vi "TreeUpdate.vi"(8 "error in":errorcluster, 11 "Data input":T1) -> (0 "error out":errorcluster, 3 "Data output":T1)   [LabVIEW 2017]
doc: "<B>This VI is used for updating tree item with Caps properties.</B>"
uses:
  Ctrl/Data.ctl
  Ctrl/Caps.ctl
  Ctrl/Property.ctl
  Ctrl/PhysicalChannel.ctl
  Ctrl/Register.ctl
  Ctrl/Bitfield.ctl
  Ctrl/Scale.ctl
  Ctrl/ScaleType.ctl
  Ctrl/Enum.ctl
  Ctrl/EnumValue.ctl
  API/Tree/SLSC Tree Control.lvlib
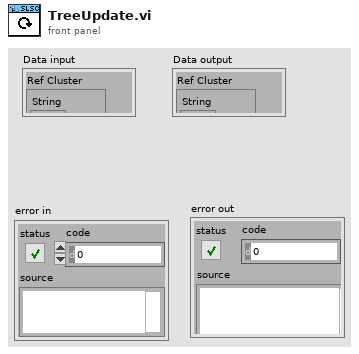
[diagram p1: front panel]
types:
  T1 = typedef "Data.ctl" = cluster{"Ref Cluster":cluster{"String":refnum<vi>, "U8":refnum<vi>, "I8":refnum<vi>, "U32":refnum<vi>, "I32":refnum<vi>, "U64":refnum<vi>, "I64":refnum<vi>, "Ring":refnum<vi>, "DBL":refnum<vi>, "Add":refnum<vi>, "Remove":refnum<vi>, "Property tree":refnum<vi>, "confirm":refnum<vi>}, "JSON Text":string, "Original JSON Text":string, "Caps":T2, "SLSC Output Tree":cluster{"Left Cell String":string, "Child Text":string[], "Child Tag":string, "Item Indent":i32, "Child Only?":bool, "Glyph Index":i32, "offline value":variant}[], "Ref Index and Control Type":cluster{"index":i32, "Datatype":string}, "Selected Type and name":cluster{"Selected Type":enum16{"Property", "Physical Channel", "Other"}, "Selected Property Name":string}, "Update whole Tree?":bool}
  T2 = typedef "Caps.ctl" = cluster{"properties":T3[], "physical channels":T4[], "registers":T5[], "scales":T7[], "enums":T9[], "productName":string}
  T3 = typedef "Property.ctl" = cluster{"name":string, "bitfield":string, "value":variant, "dataType":string, "min":variant, "max":variant, "scale":string, "access":string}
  T4 = typedef "PhysicalChannel.ctl" = cluster{"name":string, "properties":T3[]}
  T5 = typedef "Register.ctl" = cluster{"name":string, "address":i32, "size":i32, "bitfields":T6[], "initialValue":variant, "connectedProperties":string[]}
  T6 = typedef "Bitfield.ctl" = cluster{"name":string, "offset":i32, "size":i32, "signed":bool}
  T7 = typedef "Scale.ctl" = cluster{"name":string, "type":T8, "params":variant}
  T8 = typedef "ScaleType.ctl" = enum16{"NoScale", "Table", "Polynomial", "Linear"}
  T9 = typedef "Enum.ctl" = cluster{"name":string, "values":T10[]}
  T10 = typedef "EnumValue.ctl" = cluster{"name":string, "value":i32}
  T11 = cluster{"name":string, "string enums":string, "values":T10[]}[]
  T12 = cluster{"Left Cell String":string, "Child Text":string[], "Child Tag":string, "Item Indent":i32, "Child Only?":bool, "Glyph Index":i32, "offline value":variant}[]
  T13 = cluster{"Left Cell String":string, "Child Text":string[], "Child Tag":string, "Item Indent":i32, "Child Only?":bool, "Glyph Index":i32, "offline value":variant}
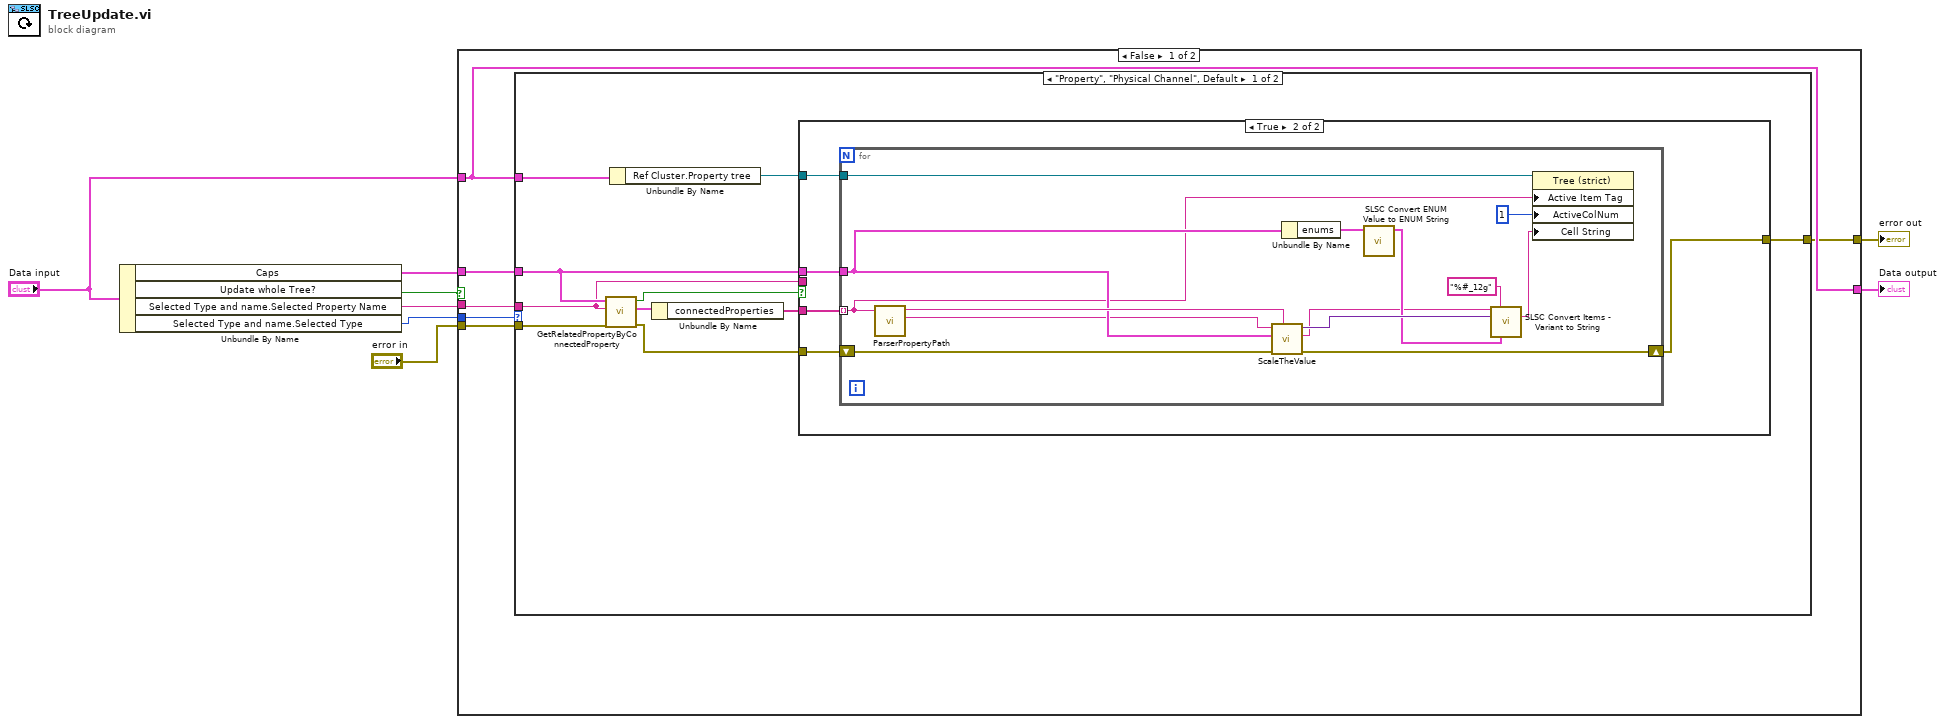
[diagram p0: block diagram]
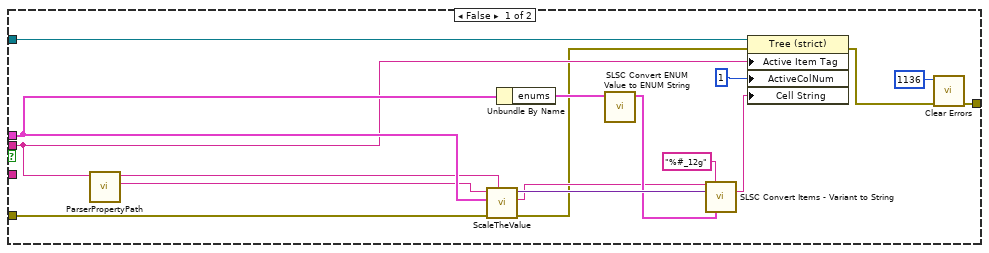
[diagram p2: hidden frame]
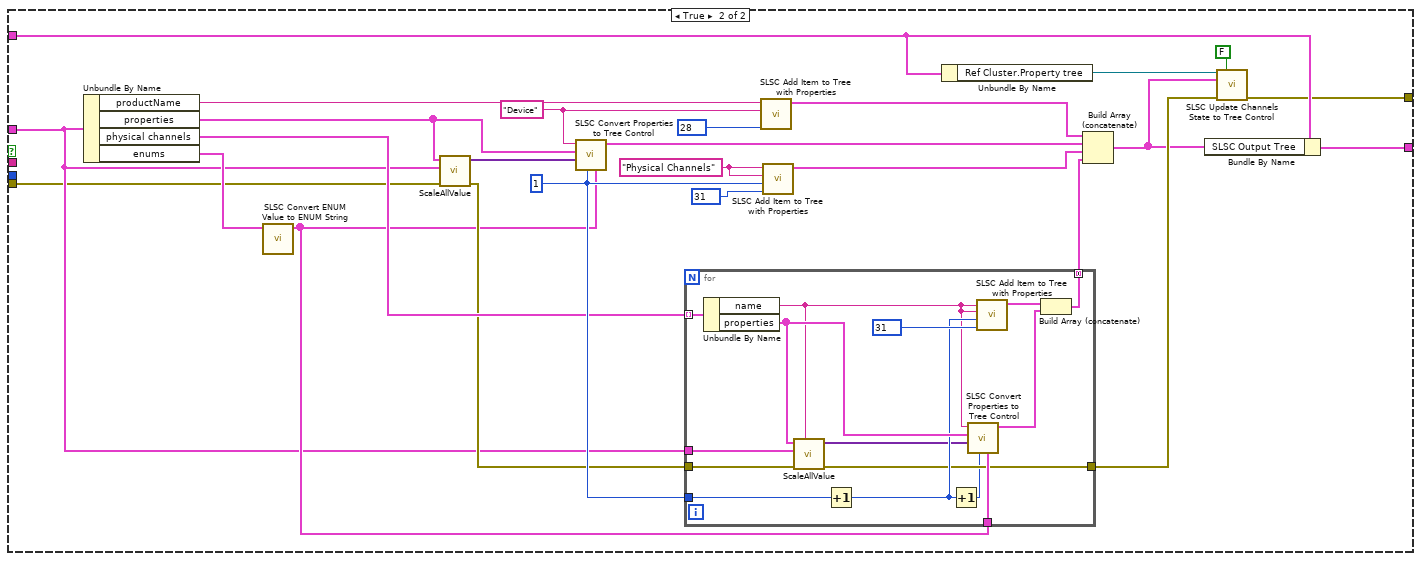
[diagram p4: hidden frame]
diagram:
  n1 = Unbundle By Name("Data input") -> ("Caps"=w7:T2, "Update whole Tree?"=w3:bool, "Selected Type and name.Selected Property Name"=w2:string, "Selected Type and name.Selected Type"=w1:enum16{"Property", "Physical Channel", "Other"})
  n2 = case shown="False" w3 {
    tunnel: [w12 w86] -> w8
    tunnel: w7 -> [w13 w65]
    tunnel: "Data input" -> [w12 w64]
    tunnel: [w11 w63] -> w5
    tunnel: w2 -> [w10 _]
    tunnel: "error in" -> [w14 w62]
    tunnel: w1 -> [w9 _]
    frame False {
      n3 = case shown="\"Property\", \"Physical Channel\", Default" w9 {
        tunnel: w14 -> [w23 w61]
        tunnel: w13 -> [w20 _]
        tunnel: w12 -> [w19 _]
        tunnel: [w17 w61] -> w11
        tunnel: w10 -> [w15 _]
        frame "Property", "Physical Channel", Default {
          n4 = call "GetRelatedPropertyByConnectedProperty.vi"("error in (no error)"=w23, "PropertyName"=w15, "Caps"=w20) -> ("error out"=w18:errorcluster, "The Register"=w24:T5, "Find?"=w16:bool)  [unwired: 5 in, 1 out]
          n5 = Unbundle By Name(w19) -> ("Ref Cluster.Property tree"=w21:refnum<vi>)
          n6 = Unbundle By Name(w24) -> ("connectedProperties"=w22:string[])
          n7 = case shown="True" w16 {
            tunnel: w22 -> [_ w46]
            tunnel: w21 -> [w41 w45]
            tunnel: w20 -> [w40 w44]
            tunnel: w18 -> [w30 w43]
            tunnel: [w26 w42] -> w17
            tunnel: w15 -> [w29 _]
            frame False {
              n8 = call "ParserPropertyPath.vi"("Seleted Item Name"=w29) -> ("Property"=w36:string, "Physical channel"=w38:string)  [unwired: 7 in]
              n9 = call "ScaleTheValue.vi"("physical channel"=w38, "error in (no error)"=w30, "Caps"=w40, "property"=w36) -> ("error out"=w28:errorcluster, "dataType"=w31:string, "offline value"=w34:variant)  [unwired: 5 in]
              n10 = Unbundle By Name(w40) -> ("enums"=w37:T9[])
              n11 = call "SLSC Convert ENUM Value to ENUM String.vi"("enums"=w37) -> ("string enums"=w33:T11)  [unwired: 10 in]
              n12 = call "SLSC Convert Items - Variant to String.vi"("dataType"=w31, "format string"="%#_12g", "value"=w34, "string enums"=w33) -> ("string offline data value"=w32:string)  [unwired: 7 in, 4 out]
              n13 = property class="Tree (strict)"(reference=w41, error in=w28, "Active Item Tag"=w29, "ActiveColNum"=1 ("Active Cell:Active Column Number"), "Cell String"=w32) -> (error out=w27:errorcluster)  [unwired: 1 out]
              n14 = call <vilib>:"Clear Errors.vi"("error in (no error)"=w27, "specific error code to clear (0: all)"=1136) -> ("error out"=w26:errorcluster)  [unwired: 4 in, 1 out]
            }
            frame True {
              n15 = for {
                tunnel: w46 -> [w47] mode=indexing
                tunnel: w45 -> [w60]
                tunnel: w44 -> [w57]
                shift-right: [w49] -> w42
                shift-left: w43 -> [w50]
                n16 = call "ParserPropertyPath.vi"("Seleted Item Name"=w47) -> ("Property"=w55:string, "Physical channel"=w58:string)  [unwired: 7 in]
                n17 = call "ScaleTheValue.vi"("physical channel"=w58, "error in (no error)"=w50, "Caps"=w57, "property"=w55) -> ("error out"=w49:errorcluster, "dataType"=w48:string, "offline value"=w53:variant)  [unwired: 5 in]
                n18 = Unbundle By Name(w57) -> ("enums"=w56:T9[])
                n19 = call "SLSC Convert ENUM Value to ENUM String.vi"("enums"=w56) -> ("string enums"=w52:T11)  [unwired: 10 in]
                n20 = call "SLSC Convert Items - Variant to String.vi"("dataType"=w48, "format string"="%#_12g", "value"=w53, "string enums"=w52) -> ("string offline data value"=w51:string)  [unwired: 7 in, 4 out]
                n21 = property class="Tree (strict)"(reference=w60, "Active Item Tag"=w47, "ActiveColNum"=1 ("Active Cell:Active Column Number"), "Cell String"=w51) -> ()  [unwired: 1 in, 2 out]
              }
            }
          }
        }
        frame "Other" {
        }
      }
    }
    frame True {
      w80 = 1
      w82 = "Physical Channels"
      w84 = "Device"
      n22 = Unbundle By Name(w65) -> ("productName"=w76:string, "properties"=w78:T3[], "physical channels"=w75:T4[], "enums"=w79:T9[])
      n23 = call "SLSC Convert ENUM Value to ENUM String.vi"("enums"=w79) -> ("string enums"=w67:T11)  [unwired: 10 in]
      n24 = call "ScaleAllValue.vi"("error in (no error)"=w62, "Caps"=w65, "properties"=w78) -> ("error out"=w68:errorcluster, "Init Value"=w77:variant[])  [unwired: 7 in]
      n25 = call "SLSC Convert Properties to Tree Control.vi"("string enums"=w67, "Item Indent"=w80, "Init Values"=w77, "properties"=w78, "Child Tag"=w84) -> ("Tree Items"=w71:T12)  [unwired: 6 in]
      n26 = for {
        tunnel: w75 -> [w101] mode=indexing
        tunnel: w68 -> [w100]
        tunnel: w67 -> [w95]
        tunnel: w80 -> [w94]
        tunnel: [w92] -> w74 mode=concatenating
        tunnel: [w91] -> w69
        tunnel: w65 -> [w90]
        n27 = Unbundle By Name(w101) -> ("name"=w89:string, "properties"=w98:T3[])
        n28 = call "ScaleAllValue.vi"("physical channel"=w89, "error in (no error)"=w100, "Caps"=w90, "properties"=w98) -> ("error out"=w91:errorcluster, "Init Value"=w88:variant[])  [unwired: 6 in]
        n29 = Increment(x=w94) -> (x+1=w93:i32)
        n30 = Increment(x=w93) -> (x+1=w87:i32)
        n31 = call "SLSC Convert Properties to Tree Control.vi"("string enums"=w95, "Item Indent"=w87, "Init Values"=w88, "properties"=w98, "Child Tag"=w89) -> ("Tree Items"=w96:T12)  [unwired: 6 in]
        n32 = call "SLSC Add Item to Tree with Properties.vi"("Glyph Index"=31, "Item indent"=w93, "Child Tag"=w89, "Left Cell String"=w89) -> ("Item"=w97:T13)  [unwired: 7 in]
        n33 = Build Array (concatenate)(w97, w96) -> (w92:T12)
      }
      n34 = call "SLSC Add Item to Tree with Properties.vi"("Glyph Index"=28, "Child Tag"=w84, "Left Cell String"=w76) -> ("Item"=w72:T13)  [unwired: 8 in]
      n35 = call "SLSC Add Item to Tree with Properties.vi"("Glyph Index"=31, "Item indent"=w80, "Child Tag"=w82, "Left Cell String"=w82) -> ("Item"=w73:T13)  [unwired: 7 in]
      n36 = Unbundle By Name(w64) -> ("Ref Cluster.Property tree"=w70:refnum<vi>)
      n37 = Build Array (concatenate)(w72, w71, w73, w74) -> (w66:T12)
      n38 = Bundle By Name(cluster=w64, "SLSC Output Tree"=w66) -> (w86:T1)
      n39 = call "SLSC Update Channels State to Tree Control.vi"("Property tree"=w70, "Update Only?"=FALSE, "SLSC Output Tree"=w66, "error in (no error)"=w69) -> ("error out"=w63:errorcluster)  [unwired: 11 in]
    }
  }
  "Data output" <- w8
  "error out" <- w5
